vi "RemoteVI Panel Controls.vi"(0 "Panel":refnum<vi>, 11 "error in":errorcluster) -> (4 "Controls":refnum<vi>[](array[refnum]), 5 "Panes":refnum<vi>[](array[refnum]), 15 "error out":errorcluster)   [LabVIEW 2020, in "RemoteVI.lvlib"]
doc: "The controls of Panel a user can see now, with the pane each one's coordinates refer to: the top-level controls of every pane (Front Panel:Controls[] with their OwningPane), then two levels inside them (RemoteVI Control Children.vi: the selected page of a tab control, cluster elements), each with the pane of the top-level control it belongs to - a cluster element's own OwningPane can name another pane (measured on a cluster moved between panes). Inner controls come first: the second level, the first, then the top level. For RemoteVI Read Tips.vi. Errors of the property reads go to error out."
uses:
  RemoteVI.lvlib
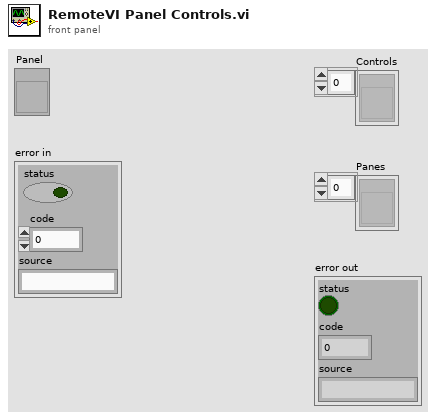
[diagram p1: front panel]
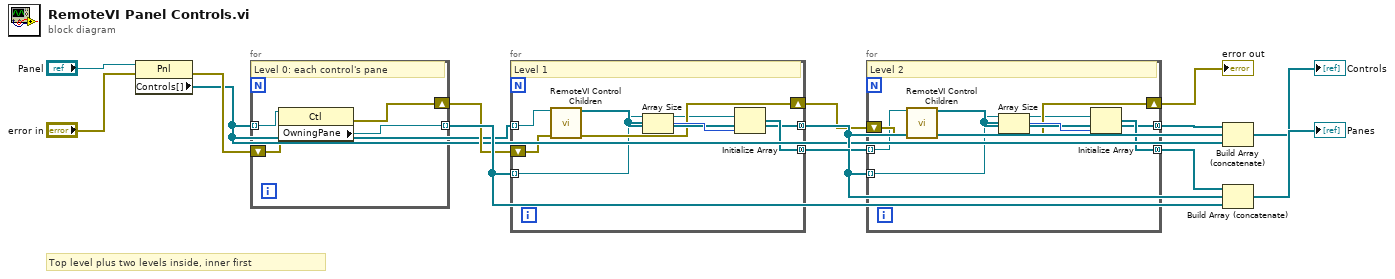
[diagram p0: block diagram]
diagram:
  # "Top level plus two levels inside, inner first"
  n1 = property class="Pnl"(reference="Panel", error in="error in") -> (error out=w4:errorcluster, "Controls[]"=w3:refnum<vi>[])  [unwired: 1 out]
  n2 = for {
    tunnel: w3 -> [w15] mode=indexing
    shift-right: [w17] -> w5
    shift-left: w4 -> [w16]
    tunnel: [w18] -> w6 mode=indexing
    # "Level 0: each control's pane"
    n3 = property class="Ctl"(reference=w15, error in=w16) -> (error out=w17:errorcluster, "OwningPane"=w18:refnum<vi>)  [unwired: 1 out]
  }
  n4 = for {
    tunnel: w3 -> [w19] mode=indexing
    shift-right: [w22] -> w7
    shift-left: w5 -> [w21]
    tunnel: w6 -> [w20] mode=indexing
    tunnel: [w23] -> w8 mode=concatenating
    tunnel: [w25] -> w9 mode=concatenating
    # "Level 1"
    n5 = call "RemoteVI Control Children.vi"("Control"=w19, "error in"=w21) -> ("Children"=w23:refnum<vi>[], "error out"=w22:errorcluster)  [unwired: 12 in]
    n6 = Array Size(array=w23) -> (size(s)=w24:i32)
    n7 = Initialize Array(w20, w24) -> (w25:refnum<vi>[])
  }
  n8 = for {
    shift-right: [w29] -> w10
    shift-left: w7 -> [w28]
    tunnel: w8 -> [w26] mode=indexing
    tunnel: w9 -> [w27] mode=indexing
    tunnel: [w30] -> w11 mode=concatenating
    tunnel: [w32] -> w12 mode=concatenating
    # "Level 2"
    n9 = call "RemoteVI Control Children.vi"("Control"=w26, "error in"=w28) -> ("Children"=w30:refnum<vi>[], "error out"=w29:errorcluster)  [unwired: 12 in]
    n10 = Array Size(array=w30) -> (size(s)=w31:i32)
    n11 = Initialize Array(w27, w31) -> (w32:refnum<vi>[])
  }
  "error out" <- w10
  n12 = Build Array (concatenate)(w11, w8, w3) -> (→"Controls":refnum<vi>[])
  n13 = Build Array (concatenate)(w12, w9, w6) -> (→"Panes":refnum<vi>[])
